vi "GServer_Constructor.vi"(6 "Debug":bool, 7 "Pane":refnum<vi>, 8 "error in (no error)":errorcluster, 9 "DAQ-Queue":refnum<queue>, 10 "Database location":path=path "G:/Sgraph_database", 11 "Gserver in":refnum<class "Gserver.lvclass">) -> (0 "error out":errorcluster, 3 "Gserver out":refnum<class "Gserver.lvclass">)   [LabVIEW 2020, in "Sgraph_lib_V1.lvlib" / "Gserver.lvclass"]
doc: "Constructor of the Gserver class."
uses:
  Gserver.lvclass
  C:/Sgraph/Sgraph/source/Vsolver/Vsolver.lvclass
  HISW/controls/typedef-DAQ-datagram.ctl
  HISW/controls/typedef-Qtype.ctl
  controls/Typedef_Gserver-init.ctl
  Gserver.lvclass/Gserver.ctl
  FAMM/FAMM.lvclass
  Common/controls/Global-services.vi
  Vsolver/Vsolver.lvclass
  Builds/Sgraph_lib_V1.lvlib
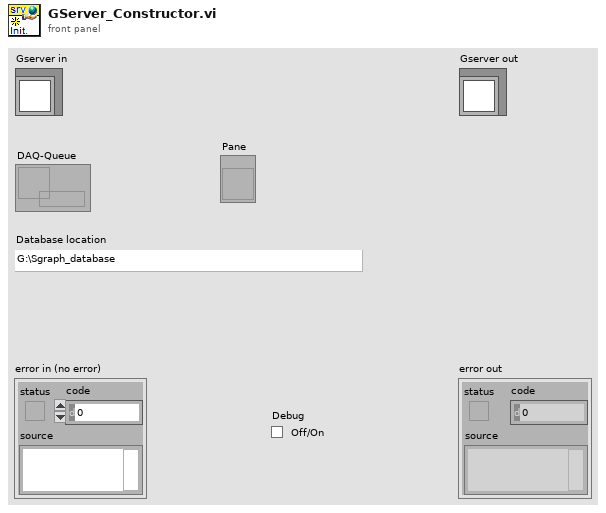
[diagram p1: front panel]
types:
  T1 = typedef "Sgraph_lib_V1.lvlib/Gserver.lvclass/Typedef_Gserver-init.ctl" = enum16{"InitStarted", "FAMM_started", "HISW_Started", "Active"}
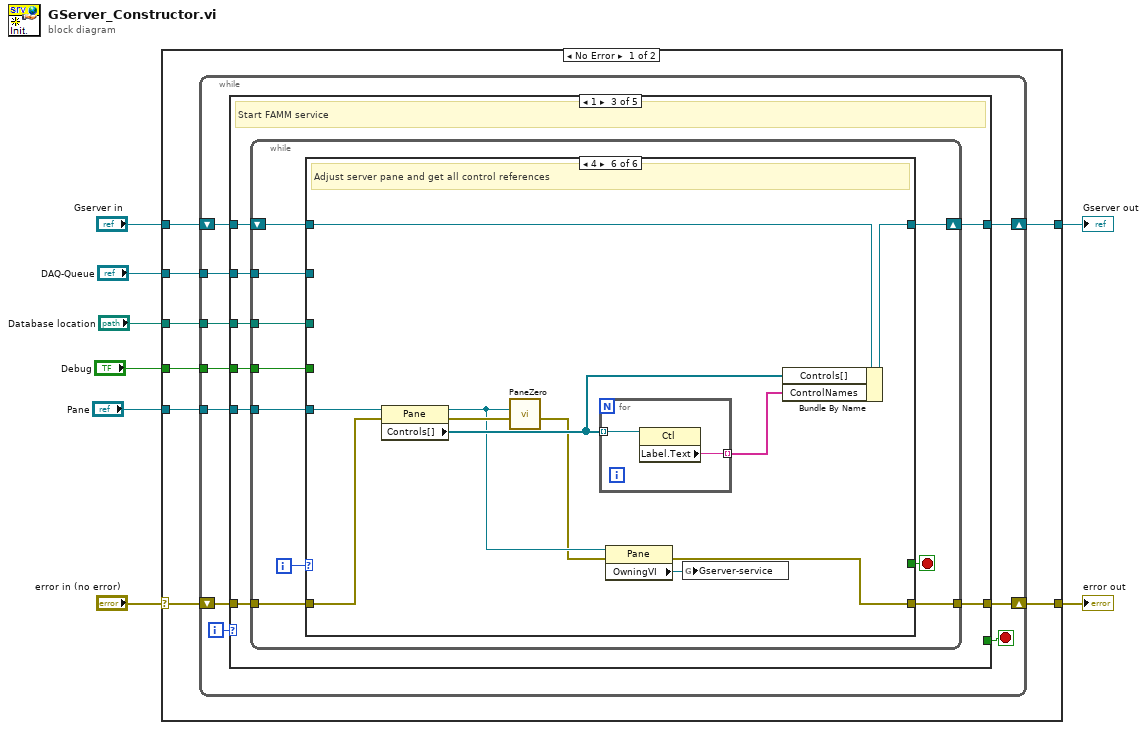
[diagram p0: block diagram]
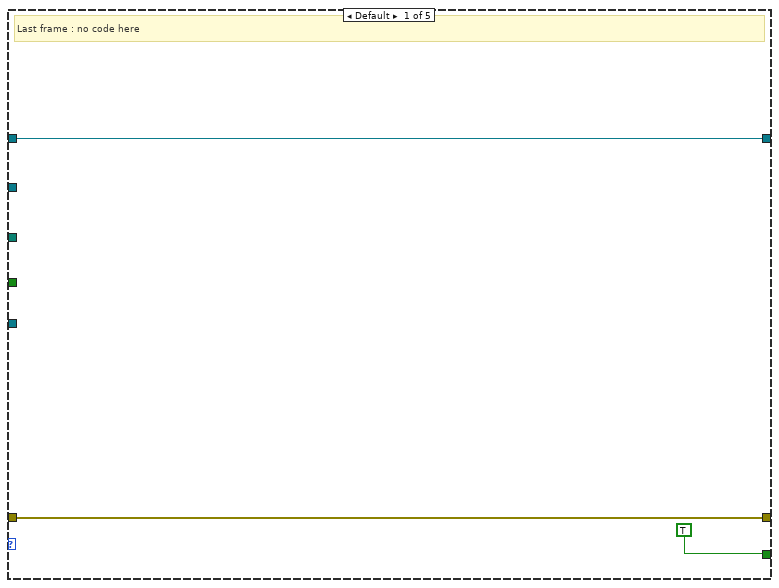
[diagram p2: hidden frame]
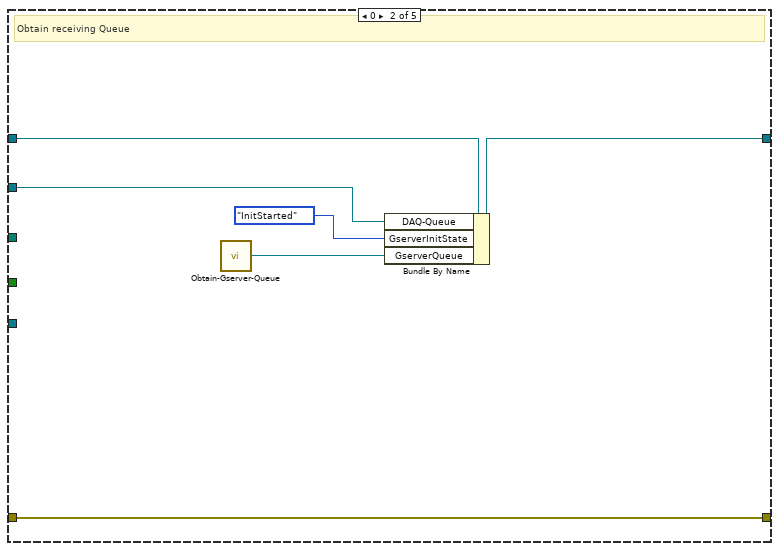
[diagram p3: hidden frame]
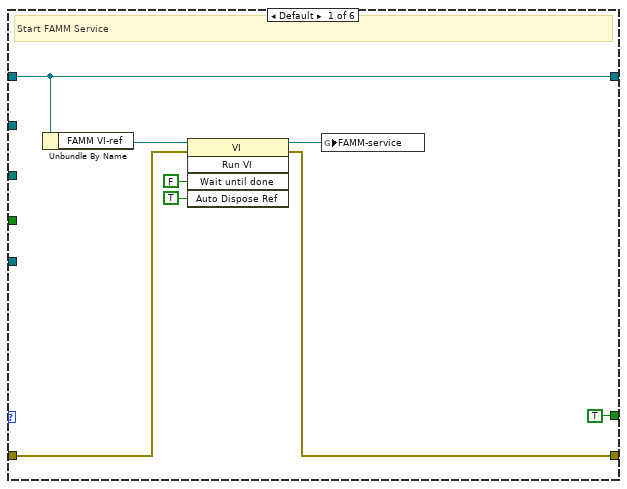
[diagram p4: hidden frame]
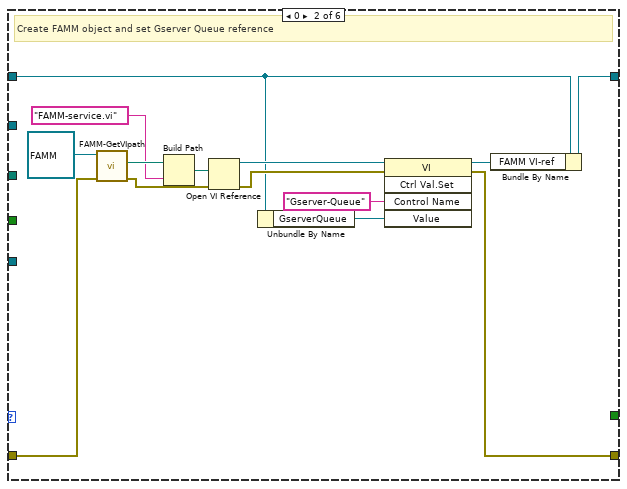
[diagram p5: hidden frame]
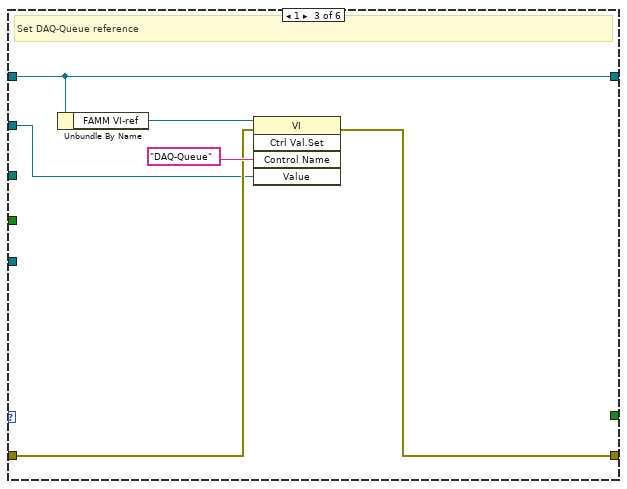
[diagram p6: hidden frame]
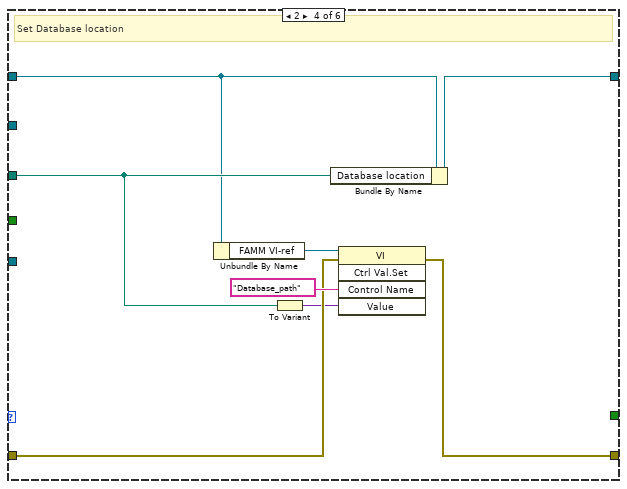
[diagram p7: hidden frame]
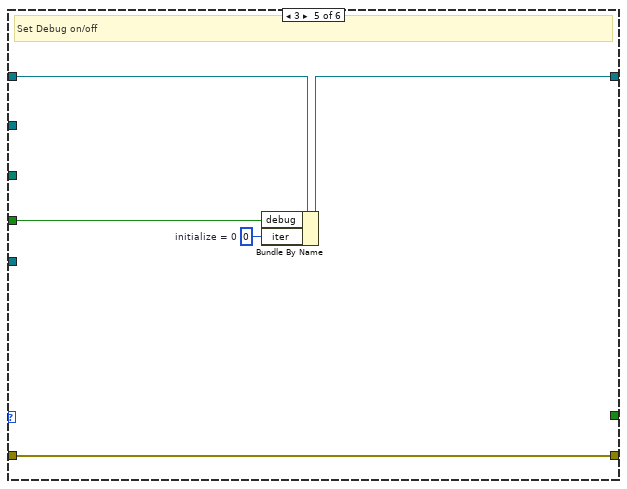
[diagram p8: hidden frame]
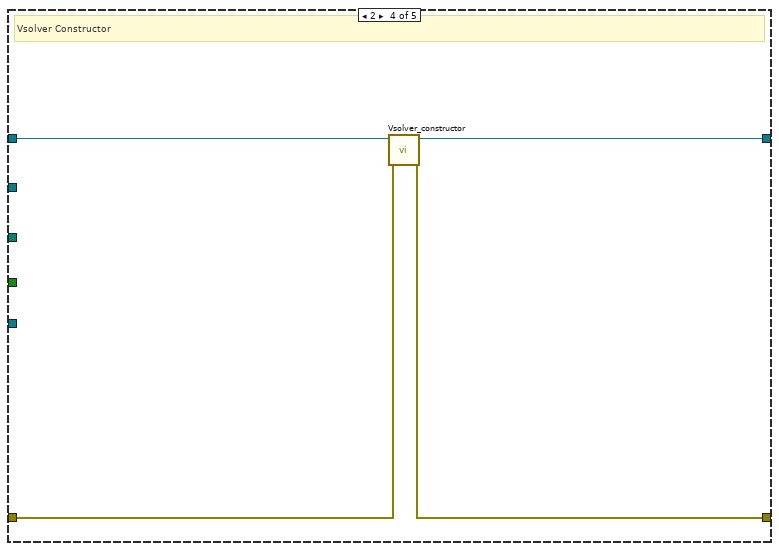
[diagram p9: hidden frame]
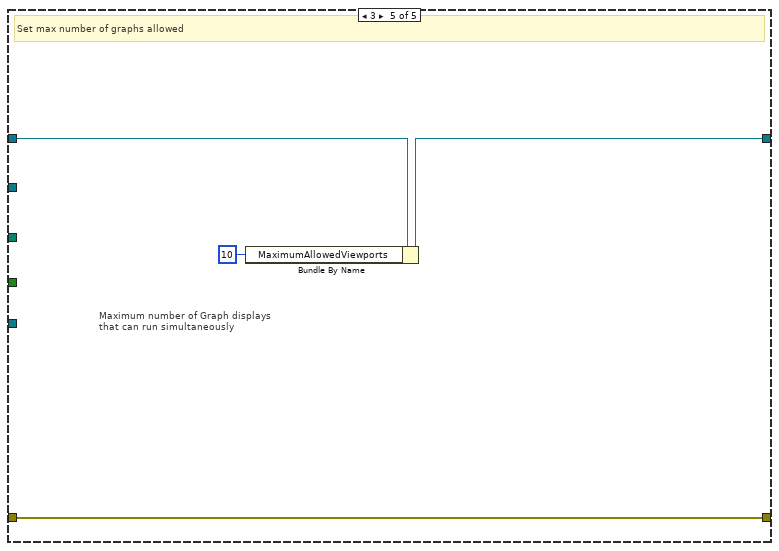
[diagram p10: hidden frame]
diagram:
  n1 = case shown="No Error" "error in (no error)" {
    selector: "error in (no error)" -> [w15 w117]
    tunnel: [w14 w117] -> w7
    tunnel: [w13 w116] -> w5
    tunnel: "Gserver in" -> [w16 w116]
    tunnel: "DAQ-Queue" -> [w12 _]
    tunnel: "Database location" -> [w11 _]
    tunnel: "Debug" -> [w10 _]
    tunnel: "Pane" -> [w9 _]
    frame No Error {
      n2 = while {
        shift-right: [w21] -> w13
        shift-left: w16 -> [w22]
        shift-right: [w23] -> w14
        shift-left: w15 -> [w26]
        tunnel: w12 -> [w20]
        tunnel: w11 -> [w19]
        tunnel: w10 -> [w18]
        tunnel: w9 -> [w17]
        i -> [w25]
        stop <- w24 stop-if-true
        n3 = case shown="1" w25 {
          tunnel: w26 -> [w28 w30 w43 w111 w112]
          tunnel: [TRUE _ _ _ _] -> w24
          tunnel: [w28 w30 w41 w110 w112] -> w23
          tunnel: w22 -> [w27 w35 w42 w109 w115]
          tunnel: [w27 w34 w38 w108 w114] -> w21
          tunnel: w20 -> [_ w32 w40 _ _]
          tunnel: w19 -> [_ _ w39 _ _]
          tunnel: w18 -> [_ _ w37 _ _]
          tunnel: w17 -> [_ _ w36 _ _]
          frame Default {
            # "Last frame : no code here"
          }
          frame 0 {
            # "Obtain receiving Queue"
            n4 = call "Obtain-Gserver-Queue.vi"() -> ("Gserver Queue"=w31:refnum<queue>)  [unwired: 7 in]
            n5 = Bundle By Name(cluster=w35, "DAQ-Queue"=w32, "GserverInitState"=Typedef_Gserver-init."InitStarted", "GserverQueue"=w31) -> (w34:refnum<class "Gserver.lvclass">)
          }
          frame 1 {
            # "Start FAMM service"
            n6 = while {
              tunnel: w43 -> [w53]
              shift-right: [w49] -> w38
              shift-left: w42 -> [w52]
              tunnel: [w46] -> w41
              tunnel: w40 -> [w48]
              tunnel: w39 -> [w47]
              tunnel: w37 -> [w45]
              tunnel: w36 -> [w44]
              i -> [w51]
              stop <- w50 stop-if-true
              n7 = case shown="4" w51 {
                tunnel: w53 -> [w56 w70 w78 w87 w94 w104]
                tunnel: w52 -> [w54 w64 w79 w82 w93 w102]
                tunnel: [TRUE _ _ _ _ _] -> w50
                tunnel: [w54 w65 w79 w83 w91 w101] -> w49
                tunnel: w48 -> [_ _ w76 _ _ _]
                tunnel: w47 -> [_ _ _ w84 _ _]
                tunnel: [w55 w62 w77 w86 w94 w95] -> w46
                tunnel: w45 -> [_ _ _ _ w92 _]
                tunnel: w44 -> [_ _ _ _ _ w105]
                frame Default {
                  # "Start FAMM Service"
                  n8 = Unbundle By Name(w54) -> ("FAMM VI-ref"=w57:refnum<vi>)
                  n9 = invoke class="VI" method="Run VI"(reference=w57, error in=w56, "Wait until done"=FALSE ("Wait Until Done"), "Auto Dispose Ref"=TRUE ("Auto Dispose Reference")) -> (reference out=w60:refnum<vi>, error out=w55:errorcluster)  [unwired: 1 in, 3 out]
                  n10 = global write "Global-services.vi" "FAMM-service"(w60) -> ()
                }
                frame 0 {
                  # "Create FAMM object and set Gserver Queue reference"
                  n11 = call "FAMM-GetVIpath.vi"("error in (no error)"=w70, "FAMM in"=refnum<class "FAMM.lvclass"> refnum ("FAMM.lvclass")) -> ("error out"=w71:errorcluster, "MethodsPath"=w74:path)  [unwired: 7 in, 1 out]
                  n12 = Build Path(base path=w74, name or relative path="FAMM-service.vi") -> (appended path=w72:path)
                  n13 = Open VI Reference(vi path=w72, error in (no error)=w71) -> (vi reference=w68:refnum<vi>, error out=w67:errorcluster)  [unwired: 4 in]
                  n14 = Unbundle By Name(w64) -> ("GserverQueue"=w66:refnum<queue>)
                  n15 = invoke class="VI" method="Ctrl Val.Set"(reference=w68, error in=w67, "Control Name"="Gserver-Queue", "Value"=w66) -> (reference out=w63:refnum<vi>, error out=w62:errorcluster)  [unwired: 1 in, 3 out]
                  n16 = Bundle By Name(cluster=w64, "FAMM VI-ref"=w63) -> (w65:refnum<class "Gserver.lvclass">)
                }
                frame 1 {
                  # "Set DAQ-Queue reference"
                  n17 = Unbundle By Name(w79) -> ("FAMM VI-ref"=w80:refnum<vi>)
                  n18 = invoke class="VI" method="Ctrl Val.Set"(reference=w80, error in=w78, "Control Name"="DAQ-Queue", "Value"=w76) -> (error out=w77:errorcluster)  [unwired: 1 in, 4 out]
                }
                frame 2 {
                  # "Set Database location"
                  n19 = Unbundle By Name(w82) -> ("FAMM VI-ref"=w88:refnum<vi>)
                  n20 = To Variant(anything=w84) -> (Variant=w85:variant)
                  n21 = Bundle By Name(cluster=w82, "Database location"=w84) -> (w83:refnum<class "Gserver.lvclass">)
                  n22 = invoke class="VI" method="Ctrl Val.Set"(reference=w88, error in=w87, "Control Name"="Database_path", "Value"=w85) -> (error out=w86:errorcluster)  [unwired: 1 in, 4 out]
                }
                frame 3 {
                  w90 = u64 0  # initialize = 0
                  # "Set Debug on/off"
                  n23 = Bundle By Name(cluster=w93, "debug"=w92, "iter"=w90) -> (w91:refnum<class "Gserver.lvclass">)
                }
                frame 4 {
                  # "Adjust server pane and get all control references"
                  n24 = property class="Pane"(reference=w105, error in=w104) -> (reference out=w97:refnum<vi>, error out=w103:errorcluster, "Controls[]"=w100:refnum<vi>[])
                  n25 = call "PaneZero.vi"("error in (no error)"=w103, "Pane"=w97) -> ("error out"=w96:errorcluster)  [unwired: 9 in]
                  n26 = for {
                    tunnel: w100 -> [w107] mode=indexing
                    tunnel: [w106] -> w99 mode=indexing
                    n27 = property class="Ctl"(reference=w107) -> ("Label.Text"=w106:string)  [unwired: 1 in, 2 out]
                  }
                  n28 = property class="Pane"(reference=w97, error in=w96) -> (error out=w95:errorcluster, "OwningVI"=w98:refnum<vi>)  [unwired: 1 out]
                  n29 = global write "Global-services.vi" "Gserver-service"(w98) -> ()
                  n30 = Bundle By Name(cluster=w102, "Controls[]"=w100, "ControlNames"=w99) -> (w101:refnum<class "Gserver.lvclass">)
                }
              }
            }
          }
          frame 2 {
            # "Vsolver Constructor"
            n31 = call "Vsolver_constructor.vi"("error in (no error)"=w111, "Vsolver in"=w109) -> ("error out"=w110:errorcluster, "Vsolver out"=w108:refnum<class "Gserver.lvclass">)  [unwired: 8 in]
          }
          frame 3 {
            # "Maximum number of Graph displays\nthat can run simultaneously"
            # "Set max number of graphs allowed"
            n32 = Bundle By Name(cluster=w115, "MaximumAllowedViewports"=u8 10) -> (w114:refnum<class "Gserver.lvclass">)
          }
        }
      }
    }
    frame Error {
    }
  }
  "error out" <- w7
  "Gserver out" <- w5
